vi "1g_development_temperature_v1.vi"() -> ()   [LabVIEW 2017]
uses:
  <vilib>/Instr/_visa.llb/VISA Configure Serial Port (Instr).vi
panel:
  out "?":cluster{dbl[], u16[]}(graph)
  # "REAL TIME FIBER OPTIC HULL MONITORING SYSTEM"
  # "COPY RIGHT : Dr Vishnu Prasad"
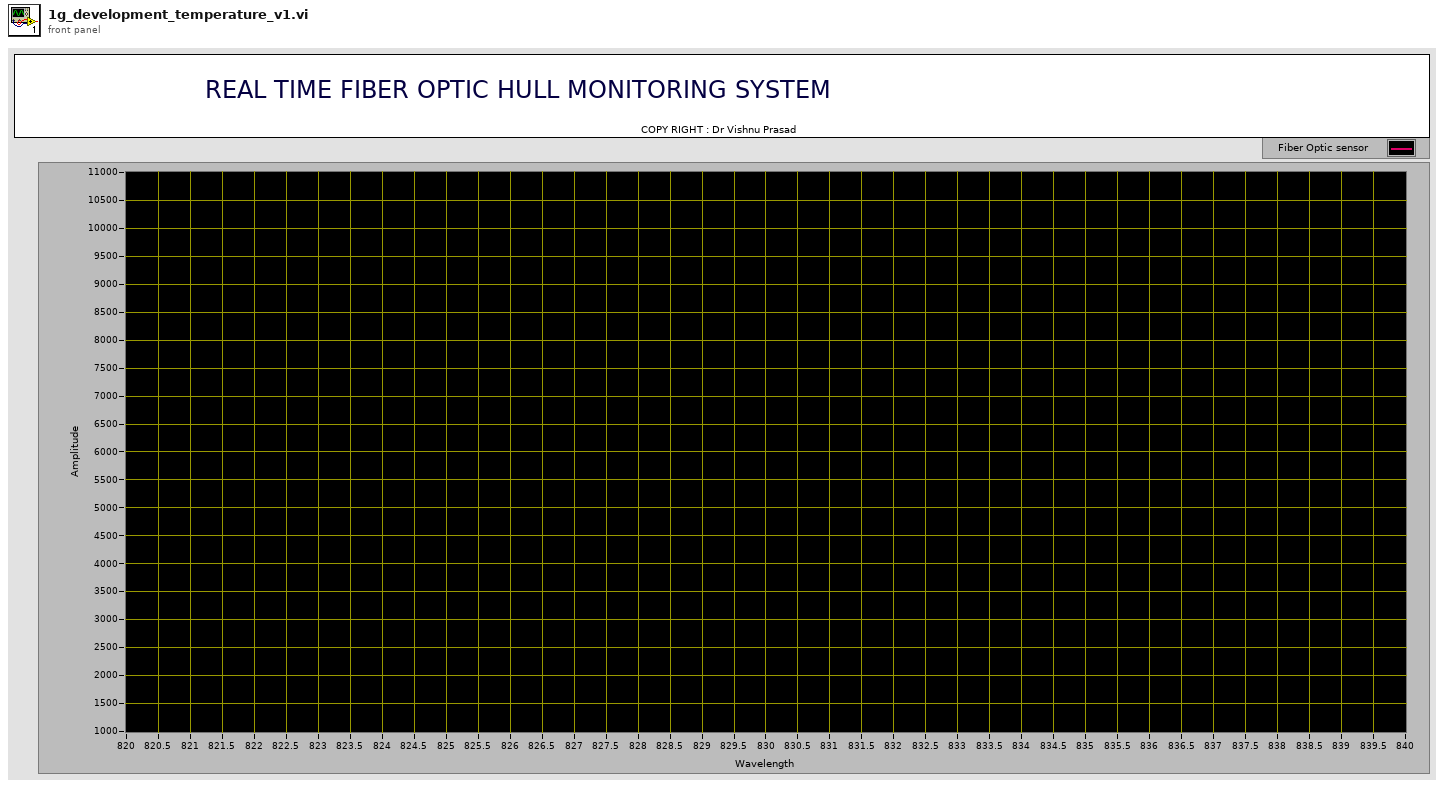
[diagram p1: front panel]
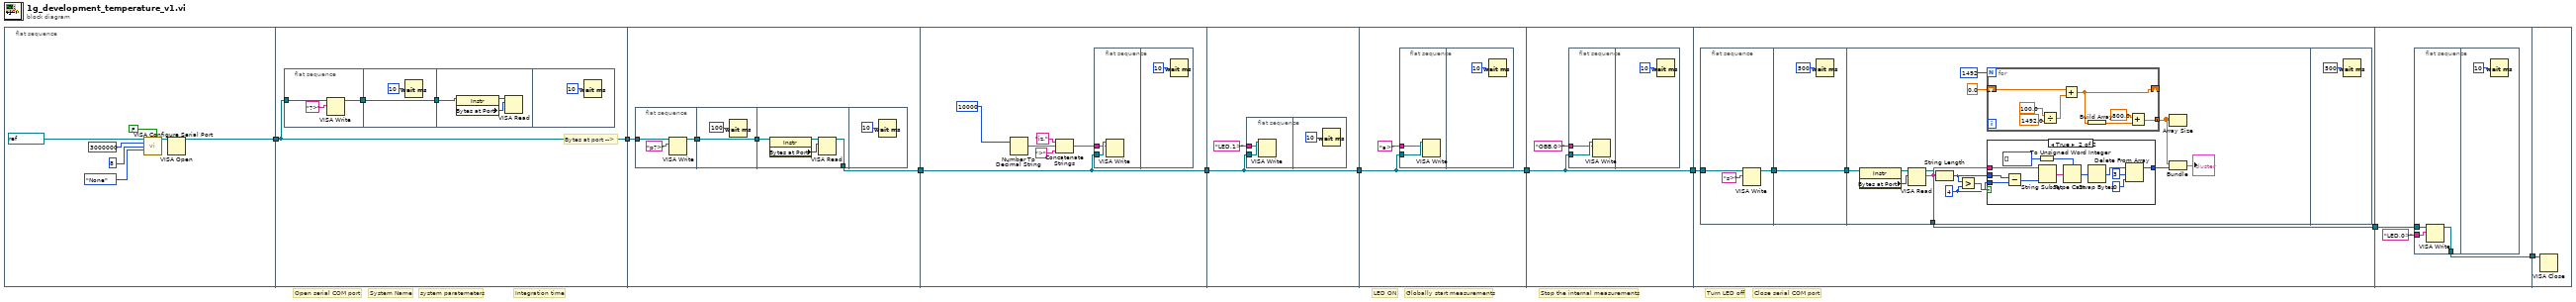
[diagram p0: block diagram]
diagram:
  # "Globally start measurements"
  # "LED ON"
  # "System Name"
  # "Integration time"
  # "system paratemeters"
  # "Close serial COM port"
  # "Turn LED off"
  # "Stop the internal measurements"
  # "Open serial COM port"
  n1 = flat-sequence {
    tunnel: [w11] -> w1
    tunnel: [w17] -> w9
    tunnel: w1 -> [w17]
    tunnel: w9 -> [w30]
    tunnel: [w29] -> w8
    tunnel: w8 -> [w44]
    tunnel: [w44] -> w7
    tunnel: w7 -> [w52]
    tunnel: [w52] -> w2
    tunnel: [w57] -> w6
    tunnel: w2 -> [w57]
    tunnel: w6 -> [w62]
    tunnel: [w62] -> w5
    tunnel: w5 -> [w68]
    tunnel: [w67] -> w4
    tunnel: w4 -> [w111]
    tunnel: [w110] -> w3
    tunnel: w3 -> [w117]
    frame #0 {
      n2 = call-poly "VISA Configure Serial Port"("VISA resource name"=refnum<visa-resource-name> "COM3", "Enable Termination\nChar (T)"=FALSE ("Enable Termination\nChar (T)"), "baud rate (9600)"=u32 3000000, "data bits (8)"=u16 8, "parity (0:none)"=enum16{"None", "Odd", "Even", "Mark", "Space"}."None") -> ("VISA resource name out"=w16:refnum<visa-resource-name>)  [unwired: 9 in, 1 out]
      n3 = VISA Open(VISA resource name=w16) -> (VISA resource name=w11:refnum<visa-resource-name>)  [unwired: 4 in, 1 out]
    }
    frame #1 {
      # "Bytes at port -->"
      n4 = flat-sequence {
        tunnel: [w22] -> w19
        tunnel: w17 -> [w21]
        tunnel: [w23] -> w18
        tunnel: w19 -> [w23]
        tunnel: w18 -> [w27]
        frame #0 {
          n5 = VISA Write(VISA resource name=w21, write buffer="?>") -> (VISA resource name out=w22:refnum<visa-resource-name>)  [unwired: 1 in, 2 out]
        }
        frame #1 {
          n6 = Wait (ms)(milliseconds to wait=u32 10 ("Zu wartende ms")) -> ()  [unwired: 1 out]
        }
        frame #2 {
          n7 = property class="Instr"(reference=w27) -> (reference out=w26:refnum<visa-resource-name>, "Bytes at Port"=w25:u32)  [unwired: 1 in, 1 out]
          n8 = VISA Read(VISA resource name=w26, byte count=w25) -> ()  [unwired: 1 in, 4 out]
        }
        frame #3 {
          n9 = Wait (ms)(milliseconds to wait=u32 10 ("Zu wartende ms")) -> ()  [unwired: 1 out]
        }
      }
    }
    frame #2 {
      n10 = flat-sequence {
        tunnel: [w35] -> w32
        tunnel: w30 -> [w33]
        tunnel: [w36] -> w31
        tunnel: w32 -> [w36]
        tunnel: w31 -> [w41]
        tunnel: [w38] -> w29
        frame #0 {
          n11 = VISA Write(VISA resource name=w33, write buffer="p?>") -> (VISA resource name out=w35:refnum<visa-resource-name>)  [unwired: 1 in, 2 out]
        }
        frame #1 {
          n12 = Wait (ms)(milliseconds to wait=u32 100 ("Zu wartende ms")) -> ()  [unwired: 1 out]
        }
        frame #2 {
          n13 = property class="Instr"(reference=w41) -> (reference out=w40:refnum<visa-resource-name>, "Bytes at Port"=w39:u32)  [unwired: 1 in, 1 out]
          n14 = VISA Read(VISA resource name=w40, byte count=w39) -> (VISA resource name out=w38:refnum<visa-resource-name>)  [unwired: 1 in, 3 out]
        }
        frame #3 {
          n15 = Wait (ms)(milliseconds to wait=u32 10 ("Zu wartende ms")) -> ()  [unwired: 1 out]
        }
      }
    }
    frame #3 {
      n16 = Number To Decimal String(number=10000) -> (decimal integer string=w48:string)  [unwired: 1 in]
      n17 = Concatenate Strings("iz," ("String"), w48, ">" ("String")) -> (w45:string)
      n18 = flat-sequence {
        tunnel: w44 -> [w50]
        tunnel: w45 -> [w49]
        frame #0 {
          n19 = VISA Write(VISA resource name=w50, write buffer=w49) -> ()  [unwired: 1 in, 3 out]
        }
        frame #1 {
          n20 = Wait (ms)(milliseconds to wait=u32 10 ("Zu wartende ms")) -> ()  [unwired: 1 out]
        }
      }
    }
    frame #4 {
      n21 = flat-sequence {
        tunnel: w52 -> [w55]
        tunnel: "LED,1>" ("String") -> [w54]
        frame #0 {
          n22 = VISA Write(VISA resource name=w55, write buffer=w54) -> ()  [unwired: 1 in, 3 out]
        }
        frame #1 {
          n23 = Wait (ms)(milliseconds to wait=u32 10 ("Zu wartende ms")) -> ()  [unwired: 1 out]
        }
      }
    }
    frame #5 {
      n24 = flat-sequence {
        tunnel: w57 -> [w60]
        tunnel: "a>" ("String") -> [w59]
        frame #0 {
          n25 = VISA Write(VISA resource name=w60, write buffer=w59) -> ()  [unwired: 1 in, 3 out]
        }
        frame #1 {
          n26 = Wait (ms)(milliseconds to wait=u32 10 ("Zu wartende ms")) -> ()  [unwired: 1 out]
        }
      }
    }
    frame #6 {
      n27 = flat-sequence {
        tunnel: w62 -> [w65]
        tunnel: "OBB,0>" ("String") -> [w64]
        frame #0 {
          n28 = VISA Write(VISA resource name=w65, write buffer=w64) -> ()  [unwired: 1 in, 3 out]
        }
        frame #1 {
          n29 = Wait (ms)(milliseconds to wait=u32 10 ("Zu wartende ms")) -> ()  [unwired: 1 out]
        }
      }
    }
    frame #7 {
      n30 = flat-sequence {
        tunnel: [w73] -> w70
        tunnel: w68 -> [w71]
        tunnel: [w74] -> w69
        tunnel: w70 -> [w74]
        tunnel: w69 -> [w83]
        tunnel: [w82] -> w67
        frame #0 {
          n31 = VISA Write(VISA resource name=w71, write buffer="s>") -> (VISA resource name out=w73:refnum<visa-resource-name>)  [unwired: 1 in, 2 out]
        }
        frame #1 {
          n32 = Wait (ms)(milliseconds to wait=u32 500 ("Zu wartende ms")) -> ()  [unwired: 1 out]
        }
        frame #2 {
          w76 = 4 ("y")
          n33 = property class="Instr"(reference=w83) -> (reference out=w81:refnum<visa-resource-name>, "Bytes at Port"=w80:u32)  [unwired: 1 in, 1 out]
          n34 = VISA Read(VISA resource name=w81, byte count=w80) -> (VISA resource name out=w82:refnum<visa-resource-name>, read buffer=w79:string)  [unwired: 1 in, 2 out]
          n35 = String Length(string=w79) -> (length=w78:i32)
          n36 = Greater?(x=w78, y=w76) -> (0:w77:bool)
          n37 = for {
            N: 1492 -> [_]
            shift-right: [w107] -> _
            shift-left: 0.0 -> [w108]
            tunnel: [w104] -> w88 mode=concatenating
            n38 = Divide(x=100.0 ("x/y"), y=1492.0) -> (x/y=w101:dbl)
            n39 = Add(x=w108, y=w101) -> (x+y=w107:dbl)
            n40 = Build Array(w107) -> (w105:dbl[])
            n41 = Add(x=800.0 ("x+y"), y=w105) -> (x+y=w104:dbl[])
          }
          n42 = case shown="True" w77 {
            tunnel: w79 -> [_ w100]
            tunnel: w78 -> [_ w99]
            tunnel: w76 -> [_ w98]
            tunnel: [_ w89] -> w86
            frame False {
            }
            frame True {
              n43 = Subtract(x=w99, y=w98) -> (x-y=w97:i32)
              n44 = To Unsigned Word Integer(number=i32[] []) -> (unsigned 16bit integer=w96:u16[])
              n45 = String Subset(string=w100, length (rest)=w97) -> (substring=w95:string)  [unwired: 1 in]
              n46 = Type Cast(type=w96, x=w95) -> (*(type *) &x=w93:u16[])
              n47 = Swap Bytes(anything=w93) -> (byte swapped=w92:u16[])
              n48 = Delete From Array(array=w92, length=3, index=0) -> (array with subset deleted=w89:u16[])  [unwired: 1 out]
            }
          }
          n49 = Array Size(array=w88) -> ()  [unwired: 1 out]
          n50 = Bundle(w88, w86) -> (→"?":cluster{dbl[], u16[]})  [unwired: 1 in]
        }
        frame #3 {
          n51 = Wait (ms)(milliseconds to wait=u32 500 ("Zu wartende ms")) -> ()  [unwired: 1 out]
        }
      }
    }
    frame #8 {
      n52 = flat-sequence {
        tunnel: w111 -> [w115]
        tunnel: "LED,0>" ("String") -> [w114]
        tunnel: [w113] -> w110
        frame #0 {
          n53 = VISA Write(VISA resource name=w115, write buffer=w114) -> (VISA resource name out=w113:refnum<visa-resource-name>)  [unwired: 1 in, 2 out]
        }
        frame #1 {
          n54 = Wait (ms)(milliseconds to wait=u32 10 ("Zu wartende ms")) -> ()  [unwired: 1 out]
        }
      }
    }
    frame #9 {
      n55 = VISA Close(VISA resource name=w117) -> ()  [unwired: 1 in, 1 out]
    }
  }
